vi "load s curve.vi"(3 "pulses":i32=500) -> (1 "Raw S Curve":u32[](graph))   [LabVIEW 2026]
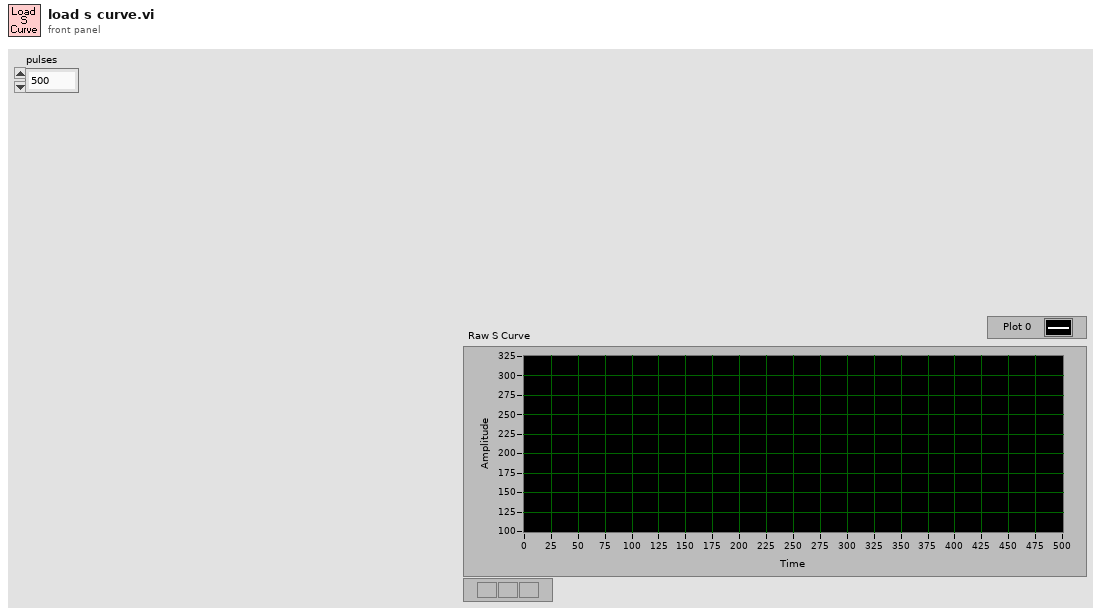
[diagram p1: front panel]
types:
  T1 = enum16{"big-endian, network order", "native, host order", "little-endian"}
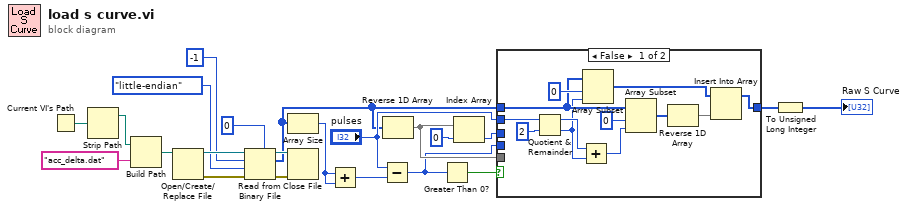
[diagram p0: block diagram]
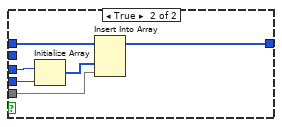
[diagram p2: hidden frame]
diagram:
  n1 = Current VI's Path() -> (path=w7:path)
  n2 = Strip Path(path=w7) -> (stripped path=w6:path)  [unwired: 1 out]
  n3 = Build Path(base path=w6, name or relative path="acc_delta.dat") -> (appended path=w4:path)
  n4 = Open/Create/Replace File(file path (use dialog)=w4) -> (refnum out=w21:refnum<file>, error out=w22:errorcluster)  [unwired: 5 in, 1 out]
  n5 = Read from Binary File(5:i16 0, 8:w22, 9:T1."little-endian" ("byte order (0:big-endian, network order)"), 10:-1 ("count (1)"), 11:w21) -> (0:w18:errorcluster, 2:w1:i16[], 3:w19:refnum<file>)  [unwired: 1 in, 1 out]
  n6 = Array Size(array=w1) -> (size(s)=w17:i32)
  n7 = Close File(refnum=w19, error in=w18) -> ()  [unwired: 2 out]
  n8 = Add(x=w17, y=w17) -> (x+y=w16:i32)
  n9 = Subtract(x="pulses", y=w16) -> (x-y=w12:i32)
  n10 = Reverse 1D Array(array=w1) -> (reversed array=w13:i16[])
  n11 = Greater Than 0?(x=w12) -> (x > 0?=w11:bool)
  n12 = Index Array(array=w13, index=0) -> (element=w14:i16)
  n13 = case shown="False" w11 {
    tunnel: w14 -> [_ w40]
    tunnel: w1 -> [w30 w39]
    tunnel: w13 -> [_ w37]
    tunnel: [w23 w36] -> w3
    tunnel: w12 -> [_ w35]
    tunnel: "pulses" -> [w33 _]
    frame False {
      n14 = Quotient & Remainder(x=w33, y=2) -> (x-y*floor(x/y)=w29:i32, floor(x/y)=w28:i32)
      n15 = Add(x=w29, y=w28) -> (x+y=w27:i32)
      n16 = Array Subset(array=w30, index=0, length=w28) -> (w25:i16[])
      n17 = Array Subset(array=w30, index=0, length=w27) -> (w26:i16[])
      n18 = Reverse 1D Array(array=w26) -> (reversed array=w24:i16[])
      n19 = Insert Into Array(array=w25, new element=w24) -> (w23:i16[])  [unwired: 1 in]
    }
    frame True {
      n20 = Initialize Array(w40, w35) -> (w38:i16[])
      n21 = Insert Into Array(array=w39, new element #1=w38, new element #2=w37) -> (w36:i16[])  [unwired: 1 in]
    }
  }
  n22 = To Unsigned Long Integer(number=w3) -> (unsigned 32bit integer=→"Raw S Curve":u32[])
